vi "Format Word for CSV.vi"(10 "data word format":T1="Hexadecimal", 11 "word":T2) -> (3 "string array":string[](array[string]))   [LabVIEW 2020, in "AIM ARINC 429 Engine.lvlib" / "Implementation.lvlib" / "CSV Word Logger.lvclass"]
uses:
  CSV Word Logger.lvclass
  Word.ctl
  Shared/Data Word Format.ctl
  Implementation.lvlib
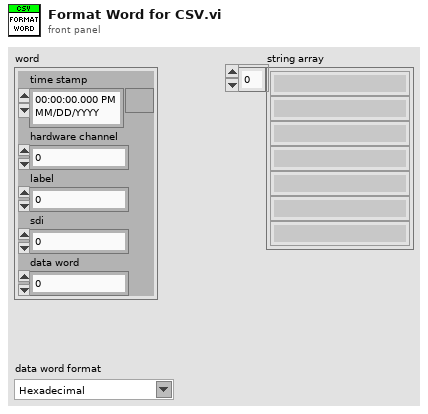
[diagram p1: front panel]
types:
  T1 = typedef "Data Word Format.ctl" = string
  T2 = typedef "AIM ARINC 429 Engine.lvlib/Implementation.lvlib/Word.ctl" = cluster{"time stamp":timestamp, "hardware channel":u8, "label":u8, "sdi":u8, "data word":u32}
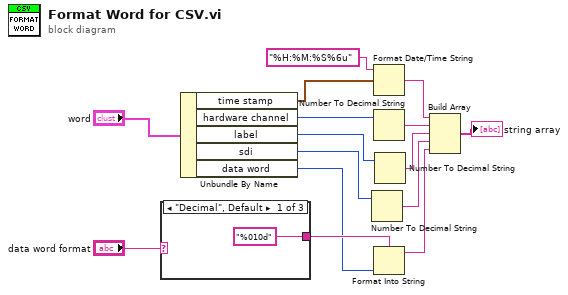
[diagram p0: block diagram]
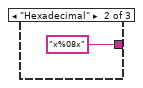
[diagram p2: hidden frame]
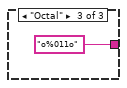
[diagram p3: hidden frame]
diagram:
  n1 = case shown="\"Decimal\", Default" "data word format" {
    tunnel: ["%010d" ("format string") "x%08x" ("format string") "o%011o" ("format string")] -> w11
    frame "Decimal", Default {
    }
    frame "Hexadecimal" {
    }
    frame "Octal" {
    }
  }
  n2 = Unbundle By Name("word") -> ("time stamp"=w10:timestamp, "hardware channel"=w14:u8, "label"=w6:u8, "sdi"=w1:u8, "data word"=w2:u32)
  n3 = Number To Decimal String(number=w1) -> (decimal integer string=w3:string)  [unwired: 1 in]
  n4 = Format Date/Time String(time format string (%c)="%H:%M:%S%6u", seconds (now)=w10) -> (date/time string=w5:string)  [unwired: 1 in]
  n5 = Number To Decimal String(number=w14) -> (decimal integer string=w8:string)  [unwired: 1 in]
  n6 = Format Into String(format string=w11, w2) -> (resulting string=w4:string)  [unwired: 2 in, 1 out]
  n7 = Number To Decimal String(number=w6) -> (decimal integer string=w7:string)  [unwired: 1 in]
  n8 = Build Array(w5, w8, w7, w3, w4) -> (→"string array":string[])
